vi "FuncVI_Sub - File - path of top-level VI in call chain.vi"() -> (0 "Top-Level VI Path":path)   [LabVIEW 2021]
doc: "::: CalcExpress Toolkit :::\nCopyright (c) 2000-2026 Konstantin Shifershteyn. All rights reserved."
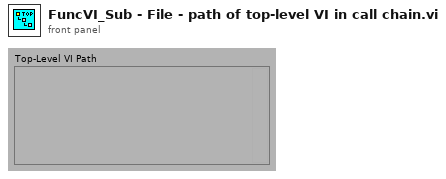
[diagram p1: front panel]
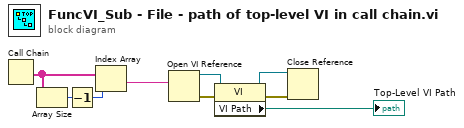
[diagram p0: block diagram]
diagram:
  n1 = Call Chain() -> (call chain=w2:string[])
  n2 = Array Size(array=w2) -> (size(s)=w3:i32)
  n3 = Decrement(x=w3) -> (x-1=w4:i32)
  n4 = Index Array(array=w2, index=w4) -> (element=w5:string)
  n5 = Open VI Reference(vi path=w5) -> (vi reference=w6:refnum<vi>, error out=w7:errorcluster)  [unwired: 5 in]
  n6 = property class="VI"(reference=w6, error in=w7) -> (reference out=w9:refnum<vi>, error out=w8:errorcluster, "VI Path"=→"Top-Level VI Path":path)
  n7 = Close Reference(reference=w9, error in (no error)=w8) -> ()  [unwired: 1 out]
